vi "Global_Init.vi"(11 "Object":T1) -> ()   [LabVIEW 2020, in "Project Provider.lvlib"]
uses:
  Project Provider.lvlib
  <resource>/Framework/Providers/API/ItemRef.ctl
  <resource>/Framework/Providers/API/mxLvMenuItem.ctl
  <resource>/Framework/Providers/API/mxLvOverlayAlias.ctl
panel:
  out "error out":errorcluster
  in  "error in":errorcluster
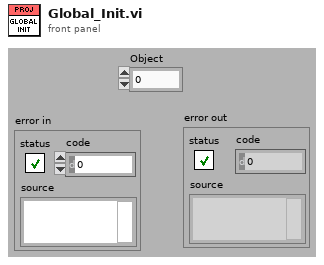
[diagram p1: front panel]
types:
  T1 = typedef "ItemRef.ctl" = u64
  T2 = typedef "mxLvMenuItem.ctl" = cluster{"Menu Name":string, "Description":string, "Icon File Name":path, "Menu Tag":string, "Enabled":bool, "Checked":bool, "Separator":bool, "Batchable":bool, "Weight":i32, "Batch Mode (Ignored if Not Batchable)":enum32{"Show If All Items Support Command", "Show If Any Items Support Command"}, "Menu Location":enum32{"<None>", "Project", "Project / Build Specifications", "Tools", "Tools / Source Control", "Tools / Real-Time Module", "Help"}, "Exclude From Getting Started Window Menu":bool}
  T3 = typedef "mxLvOverlayAlias.ctl" = cluster{"Overlay Alias":string, "Icon File Name":path}
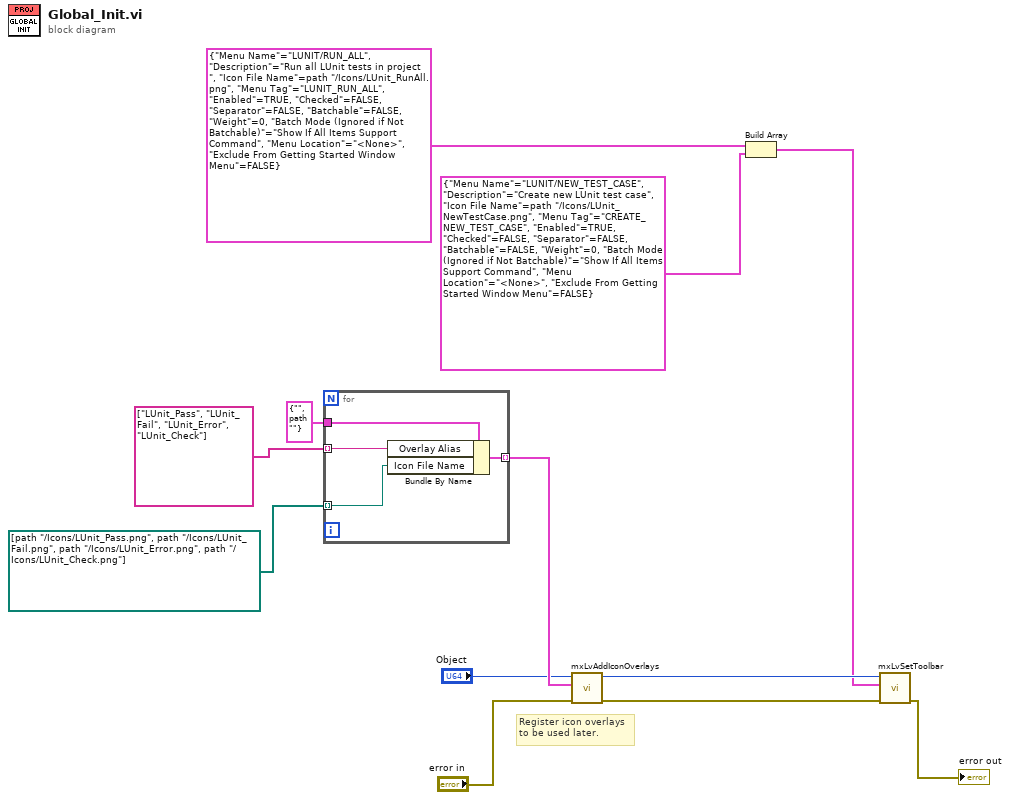
[diagram p0: block diagram]
diagram:
  # "Register icon overlays\nto be used later."
  n1 = for {
    tunnel: T3 {"Overlay Alias"="", "Icon File Name"=path ""} ("Icon Overlay Alias") -> [w16]
    tunnel: [w15] -> w11 mode=indexing
    tunnel: string[] ["LUnit_Pass", "LUnit_Fail", "LUnit_Error", "LUnit_Check"] ("overlay alias") -> [w14] mode=indexing
    tunnel: path[] [path "../Icons/LUnit_Pass.png", path "../Icons/LUnit_Fail.png", path "../Icons/LUnit_Error.png", path "../Icons/LUnit_Check.png"] ("icon filename") -> [w13] mode=indexing
    n2 = Bundle By Name(cluster=w16, "Overlay Alias"=w14, "Icon File Name"=w13) -> (w15:T3)
  }
  n3 = call <resource>:"mxLvAddIconOverlays.vi"("error in"="error in", "Overlay Aliases"=w11, "Item"="Object") -> ("error out"=w5:errorcluster, "Item"=w6:T1)  [unwired: 7 in]
  n4 = Build Array(T2 {"Menu Name"="LUNIT/RUN_ALL", "Description"="Run all LUnit tests in project ", "Icon File Name"=path "../Icons/LUnit_RunAll.png", "Menu Tag"="LUNIT_RUN_ALL", "Enabled"=TRUE, "Checked"=FALSE, "Separator"=FALSE, "Batchable"=FALSE, "Weight"=0, "Batch Mode (Ignored if Not Batchable)"=enum."Show If All Items Support Command", "Menu Location"=enum."<None>", "Exclude From Getting Started Window Menu"=FALSE} ("Menu Item"), T2 {"Menu Name"="LUNIT/NEW_TEST_CASE", "Description"="Create new LUnit test case", "Icon File Name"=path "../Icons/LUnit_NewTestCase.png", "Menu Tag"="CREATE_NEW_TEST_CASE", "Enabled"=TRUE, "Checked"=FALSE, "Separator"=FALSE, "Batchable"=FALSE, "Weight"=0, "Batch Mode (Ignored if Not Batchable)"=enum."Show If All Items Support Command", "Menu Location"=enum."<None>", "Exclude From Getting Started Window Menu"=FALSE} ("Menu Item")) -> (w2:T2[])
  n5 = call <resource>:"mxLvSetToolbar.vi"("error in"=w5, "Toolbar Items"=w2, "Item"=w6) -> ("error out"=→"error out":errorcluster)  [unwired: 7 in, 1 out]
